vi "CIVI Set Frequency.vi"(8 "error in (no error)":errorcluster, 10 "Frequency Setpoint (Hz)":i32, 11 "VISA Session in":refnum<visa-resource-name>) -> (0 "error out":errorcluster, 3 "VISA Session out":refnum<visa-resource-name>)   [LabVIEW 2026]
doc: "Formats and sends SENS:FREQ with an integer frequency in Hz.\nSends the command only.\nDoes not perform readback or query the instrument error queue.\nUse CIVI Read Frequency Session.vi and CIVI Error Query.vi\nto verify the result."
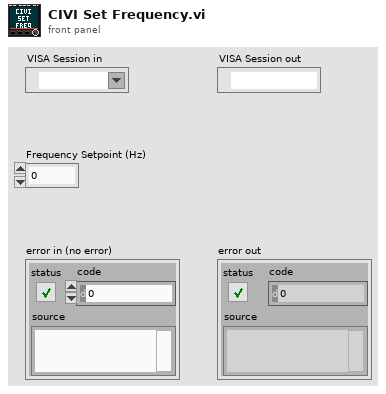
[diagram p1: front panel]
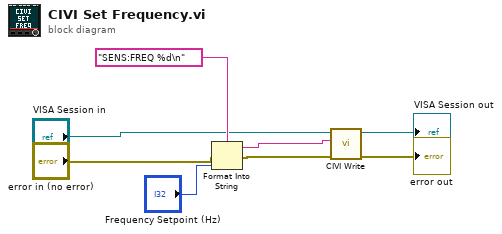
[diagram p0: block diagram]
diagram:
  n1 = Format Into String(format string="SENS:FREQ %d\n", error in="error in (no error)", "Frequency Setpoint (Hz)") -> (resulting string=w6:string, error out=w8:errorcluster)  [unwired: 1 in]
  n2 = call "CIVI Write.vi"("error in"=w8, "write buffer"=w6, "VISA Session in"="VISA Session in") -> ("error out"=→"error out":errorcluster, "VISA Session out"=→"VISA Session out":refnum<visa-resource-name>)  [unwired: 7 in]
